vi "Index Group.vi"(6 "Don't Create":bool, 8 "error in (no error)":errorcluster, 10 "Group":string, 11 "bt_Blackboard in":refnum<class "Blackboard.lvclass">) -> (0 "error out":errorcluster, 2 "Index":i32, 3 "bt_Blackboard out":refnum<class "Blackboard.lvclass">)   [LabVIEW 2021, in "Blackboard.lvclass"]
uses:
  Blackboard.lvclass
  Blackboard.lvclass/Blackboard.ctl
  Data DVR Type.ctl
  Tags Map Type.ctl
  <vilib>/TSA/Abstract Data Classes/Abs_Types/Value/Abs_Value.lvclass
  <vilib>/TSA/Omni-Bus/Local Bus/Support/Data Value References.ctl
  <vilib>/TSA/Abstract Data Classes/Abs_Types/Type/Abs_Type.lvclass
  <vilib>/TSA/Omni-Bus/Local Bus/Local Bus.lvclass
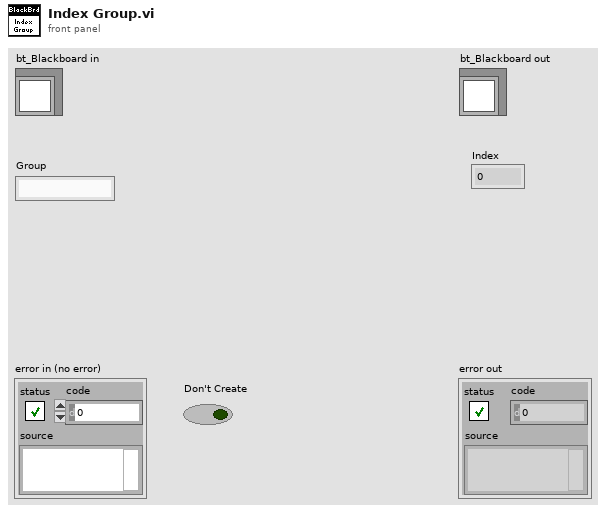
[diagram p1: front panel]
types:
  T1 = typedef "Blackboard.lvclass/Data DVR Type.ctl" = cluster{"Tags":T2, "Data Refs":T3}
  T2 = typedef "Blackboard.lvclass/Tags Map Type.ctl" = map{string, refnum<class "Abs_Value.lvclass">}
  T3 = typedef "Local Bus.lvclass/Data Value References.ctl" = cluster{"Boolean":refnum<data-value>, "String":refnum<data-value>, "DBL":refnum<data-value>, "SGL":refnum<data-value>, "EXT":refnum<data-value>, "U8":refnum<data-value>, "U16":refnum<data-value>, "U32":refnum<data-value>, "U64":refnum<data-value>, "I8":refnum<data-value>, "I16":refnum<data-value>, "I32":refnum<data-value>, "I64":refnum<data-value>, "CDBL":refnum<data-value>, "CSGL":refnum<data-value>, "CEXT":refnum<data-value>, "Time":refnum<data-value>, "Variant":refnum<data-value>, "Waveform":refnum<data-value>, "Type":refnum<data-value>}
  T4 = typedef "Blackboard.lvclass/Groups Type.ctl" = cluster{"Data":T1[], "Map":T5}
  T5 = typedef "Blackboard.lvclass/Group Map Type.ctl" = map{string, i32}
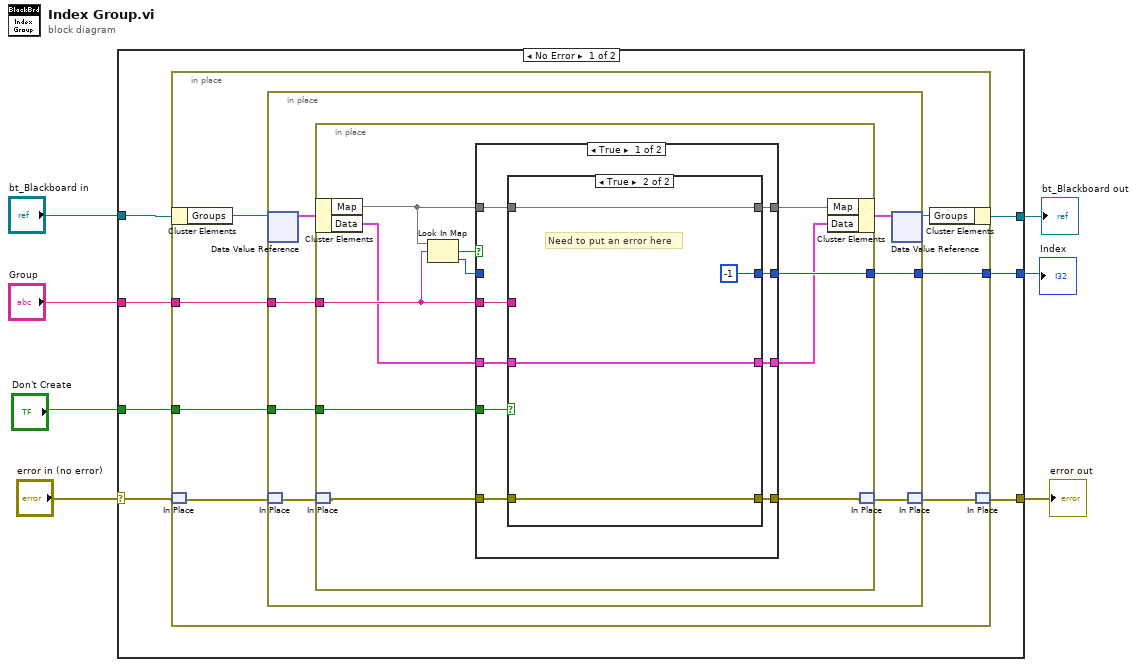
[diagram p0: block diagram]
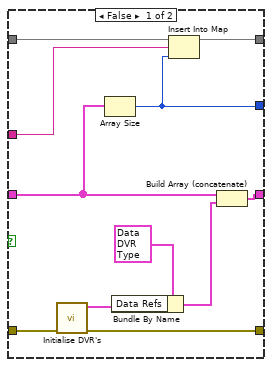
[diagram p2: hidden frame]
diagram:
  n1 = case shown="No Error" "error in (no error)" {
    selector: "error in (no error)" -> [w10 w69]
    tunnel: [w9 w69] -> w6
    tunnel: [w12 w68] -> w4
    tunnel: "bt_Blackboard in" -> [w14 w68]
    tunnel: "Group" -> [w13 _]
    tunnel: [w11 _] -> w2
    tunnel: "Don't Create" -> [w8 _]
    frame No Error {
      n2 = in-place {
        in-place-border: w13 -> [w20]
        in-place-border: [w21] -> w11
        in-place-border: w8 -> [w15]
        n3 = in-place-cluster #1(w14) -> ("Groups"=w19:refnum<data-value>)
        n4 = in-place-match #2(w10) -> (w17:errorcluster)
        n5 = in-place {
          in-place-border: [w28] -> w21
          in-place-border: w20 -> [w27]
          in-place-border: w15 -> [w22]
          n6 = in-place-dvr #3(w19) -> (w26:T4)  [unwired: 1 out]
          n7 = in-place-match #4(w17) -> (w24:errorcluster)
          n8 = in-place {
            in-place-border: [w39] -> w28
            in-place-border: w27 -> [w38]
            in-place-border: w22 -> [w29]
            n9 = in-place-cluster #5(w26) -> ("Map"=w35:T5, "Data"=w33:T1[])
            n10 = in-place-match #6(w24) -> (w31:errorcluster)
            n11 = Look In Map(map=w35, key=w38) -> (key not found?=w37:bool, value=w36:i32)  [unwired: 1 in]
            n12 = case shown="True" w37 {
              tunnel: w38 -> [w45 _]
              tunnel: [w44 w65] -> w39
              tunnel: w33 -> [w41 w67]
              tunnel: [w48 w67] -> w32
              tunnel: w31 -> [w43 w66]
              tunnel: [w42 w66] -> w30
              tunnel: w35 -> [w47 w64]
              tunnel: [w46 w64] -> w34
              tunnel: w36 -> [_ w65]
              tunnel: w29 -> [w40 _]
              frame True {
                n13 = case shown="True" w40 {
                  tunnel: [w59 w61] -> w48
                  tunnel: w47 -> [w58 w63]
                  tunnel: [w57 w63] -> w46
                  tunnel: w45 -> [w56 _]
                  tunnel: [w55 -1] -> w44
                  tunnel: w43 -> [w54 w60]
                  tunnel: [w53 w60] -> w42
                  tunnel: w41 -> [w49 w61]
                  frame False {
                    n14 = call <vilib>:"Initialise DVR's.vi"("error in (no error)"=w54) -> ("error out"=w53:errorcluster, "Data Value References"=w51:T3)  [unwired: 9 in]
                    n15 = Array Size(array=w49) -> (size(s)=w55:i32)
                    n16 = Bundle By Name(cluster=T1 {"Tags"={}, "Data Refs"={"Boolean"=refnum, "String"=refnum, "DBL"=refnum, "SGL"=refnum, "EXT"=refnum, "U8"=refnum, "U16"=refnum, "U32"=refnum, "U64"=refnum, "I8"=refnum, "I16"=refnum, "I32"=refnum, "I64"=refnum, "CDBL"=refnum, "CSGL"=refnum, "CEXT"=refnum, "Time"=refnum, "Variant"=refnum, "Waveform"=refnum, "Type"=refnum}} ("Data"), "Data Refs"=w51) -> (w50:T1)
                    n17 = Insert Into Map(map in=w58, key=w56, value=w55) -> (map out=w57:T5)  [unwired: 2 out]
                    n18 = Build Array (concatenate)(w49, w50) -> (w59:T1[])
                  }
                  frame True {
                    # "Need to put an error here"
                  }
                }
              }
              frame False {
              }
            }
            n19 = in-place-cluster #5("Map"=w34, "Data"=w32) -> (w25:T4)
            n20 = in-place-match #6(w30) -> (w23:errorcluster)
          }
          n21 = in-place-dvr #3(w25) -> (w18:refnum<data-value>)  [unwired: 1 out]
          n22 = in-place-match #4(w23) -> (w16:errorcluster)
        }
        n23 = in-place-cluster #1("Groups"=w18) -> (w12:refnum<class "Blackboard.lvclass">)
        n24 = in-place-match #2(w16) -> (w9:errorcluster)
      }
    }
    frame Error {
    }
  }
  "error out" <- w6
  "bt_Blackboard out" <- w4
  "Index" <- w2
